vi "Main.vi"(11 "Module Admin":refnum<class "Delacor_lib_QMH_Cloneable Module Admin.lvclass">) -> ()   [LabVIEW 2026, in "Function Generator.lvlib"]
doc: "This template is based off of the Queued Message Handler design pattern and the Queued Message Handler project template that ships with LabVIEW.\n\nThe main difference is that the queue is private to this module and communication between modules is performed via Broadcast and Request events.\n\nRequest events are wrapped in public API methods and are handled in the Event Handling Loop (EHL) of this VI. Any module can register for Broadcast events sent by this module. The EHL generates messages based on user interface actions.\n\nThe Message Handling Loop (MHL) processes messages generated by the EHL, or by other messages. The messages are string values, so new messages can be added easily to the Message Cases case structure in the MHL. Each message cluster can also provide an optional value for Message Data, which is a variant that can be converted to whatever message-specific data is required.\n_____\nBased on DQMH Dev Tools: Project Template 7.1.2.1547."
uses:
  Function Generator.lvlib
  <vilib>/Delacor/Delacor QMH/Libraries/Cloneable Module Admin_class/Delacor_lib_QMH_Cloneable Module Admin.lvclass
  C:/Program Files/National Instruments/LabVIEW 2026/vi.lib/Delacor/Delacor QMH/Libraries/Module Admin_class/Delacor_lib_QMH_Module Admin.lvclass
  Module Data--cluster.ctl
  <vilib>/Delacor/Delacor QMH/Libraries/Cloneable Module Admin_class/Delacor_lib_QMH_Cloneable Module Admin.lvclass/Delacor_lib_QMH_Cloneable Module Admin.ctl
  Wake Up HL Argument--cluster.ctl
  <vilib>/Delacor/Delacor QMH/Libraries/Message Queue_class/Delacor_lib_QMH_Message Queue.lvclass/Delacor_lib_QMH_Message Queue.ctl
  Stop Argument--cluster.ctl
  <vilib>/Delacor/Delacor QMH/Libraries/Module Admin_class/Delacor_lib_QMH_Module Admin.lvclass/Delacor_lib_QMH_Module Admin.ctl
  Set Signal Type Argument--cluster.ctl
  Set Signal Parameters Argument--cluster.ctl
  Start Argument--cluster.ctl
  <vilib>/Utility/miscctls.llb/LVPointTypeDef.ctl
  <vilib>/Delacor/Delacor QMH/Libraries/Cloneable Module Admin_class/Delacor_lib_QMH_Get Module ID.vi
  <vilib>/Delacor/Delacor QMH/Libraries/Message Queue_class/Delacor_lib_QMH_Enqueue Message (Single).vi
  <vilib>/Delacor/Delacor QMH/Libraries/Module Admin_class/Delacor_lib_QMH_Get External Launch.vi
  <vilib>/Delacor/Delacor QMH/Libraries/Message Queue_class/Delacor_lib_QMH_Message Queue.lvclass
  <vilib>/measure/NI_MABase.lvlib
panel:
  out "error out":errorcluster
  out "Status":string
  in  "Simulate EHL Error":bool
  in  "Simulate MHL Error":bool
  # "Other processes communicate with this Module via its Public API (wrappers for its Request Events).\n\nThis Module communicates with other processes via its Broadcast Events.\nAny process that wants to receive these messages can register for this module's Broadcast events."
  # "This template is for the DQMH framework. See the block diagram for more information on how to use this template."
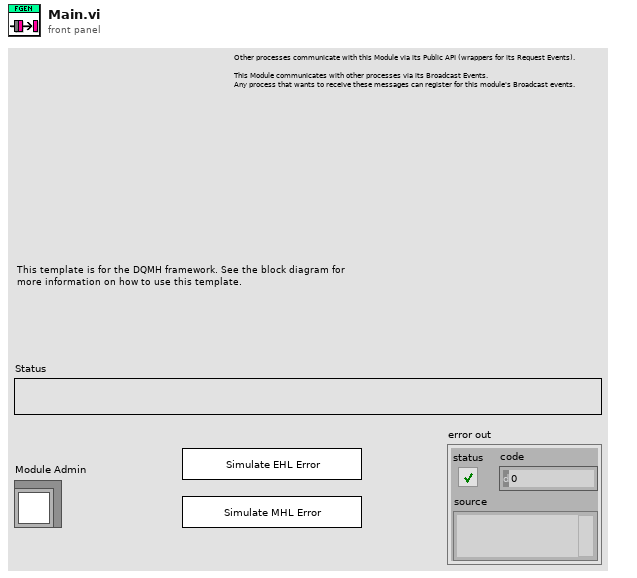
[diagram p1: front panel]
types:
  T1 = typedef "Function Generator.lvlib/Request Events--cluster.ctl" = cluster{"Stop Module":refnum<user-event>, "Show Panel":refnum<user-event>, "Hide Panel":refnum<user-event>, "Show Diagram":refnum<user-event>, "Get Module Execution Status":refnum<user-event>, "Set Signal Type":refnum<user-event>, "Set Signal Parameters":refnum<user-event>, "Start":refnum<user-event>, "Local Instance":T2, "Stop FGEN":refnum<user-event>}
  T2 = typedef "Function Generator.lvlib/Local Instance Request Events--cluster.ctl" = cluster{"Wake Up HL":refnum<user-event>}
  T3 = typedef "Function Generator.lvlib/Module Data--cluster.ctl" = cluster{"Status":string, "signal type":enum16{"Sine Wave", "Triangle Wave", "Square Wave", "Sawtooth Wave"}, "amplitude":dbl, "phase":dbl, "frequency":dbl, "offset 2":dbl}
  T4 = typedef "Function Generator.lvlib/Wake Up HL Argument--cluster.ctl" = cluster{"Module ID":i32, "Timeout":i32, "signal type":enum16{"Sine Wave", "Triangle Wave", "Square Wave", "Sawtooth Wave"}, "amplitude":dbl, "phase":dbl, "frequency":dbl, "offset 2":dbl}
  T5 = enum32{"invalid lock state", "Not Locked", "Locked (No Password)", "Password-protected"}
  T6 = typedef "Function Generator.lvlib/Stop Argument--cluster.ctl" = cluster{"Module ID":i32, "Origin":string, "Exit via Stop Module Req?":bool, "Wait for Module to stop?":bool}
  T7 = typedef "Function Generator.lvlib/Set Signal Type Argument--cluster.ctl" = cluster{"Module ID":i32, "signal type":enum16{"Sine Wave", "Triangle Wave", "Square Wave", "Sawtooth Wave"}}
  T8 = typedef "Function Generator.lvlib/Set Signal Parameters Argument--cluster.ctl" = cluster{"Module ID":i32, "amplitude":dbl, "phase":dbl, "frequency":dbl, "offset":dbl}
  T9 = typedef "Function Generator.lvlib/Start Argument--cluster.ctl" = cluster{"Module ID":i32, "Boolean":bool}
  T10 = typedef "LVPointTypeDef.ctl" = cluster{"Horizontal":i16, "Vertical":i16}
  T11 = enum32{"Invalid", "Standard", "Closed", "Hidden", "Minimized", "Maximized"}
  T12 = enum16{"Sine Wave", "Triangle Wave", "Square Wave", "Sawtooth Wave"}
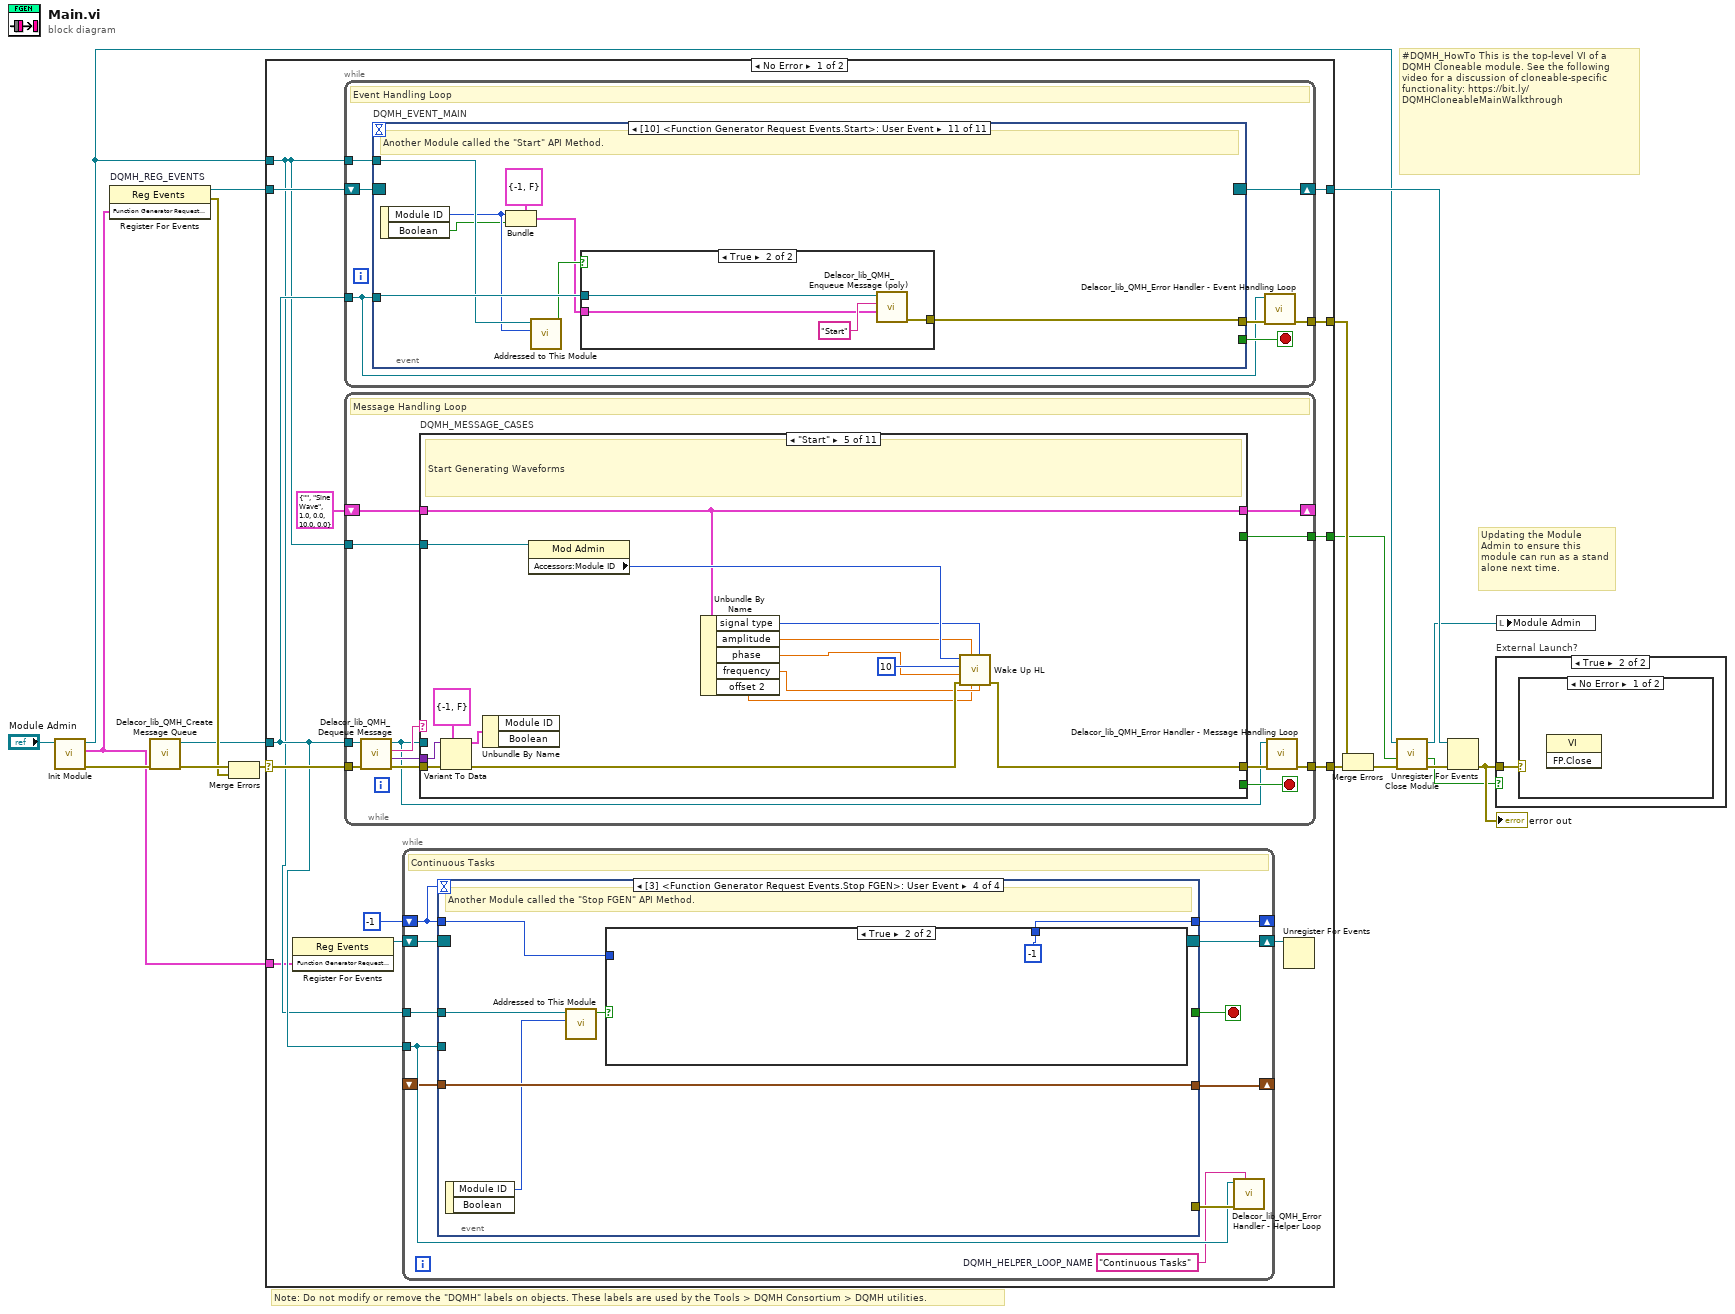
[diagram p0: block diagram]
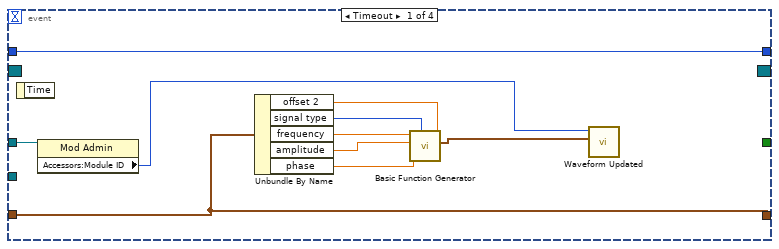
[diagram p2: hidden frame]
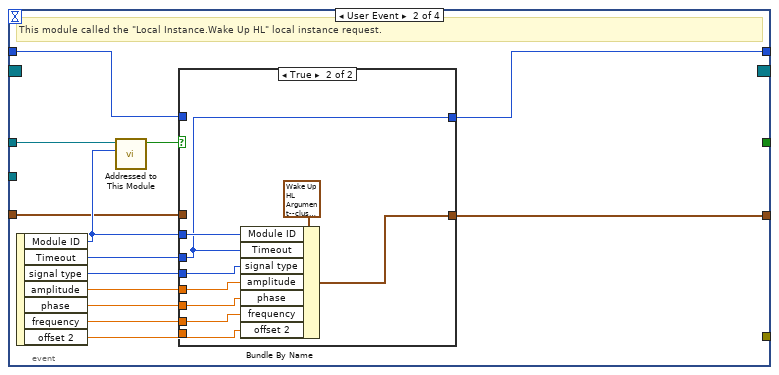
[diagram p3: hidden frame]
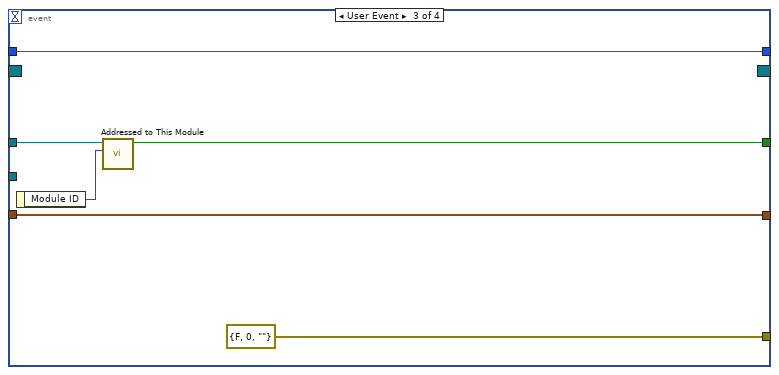
[diagram p5: hidden frame]
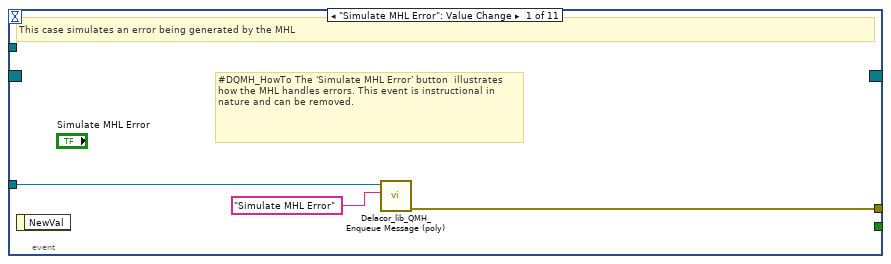
[diagram p7: hidden frame]
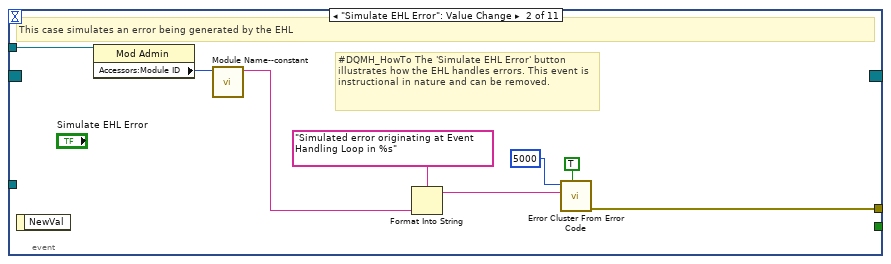
[diagram p8: hidden frame]
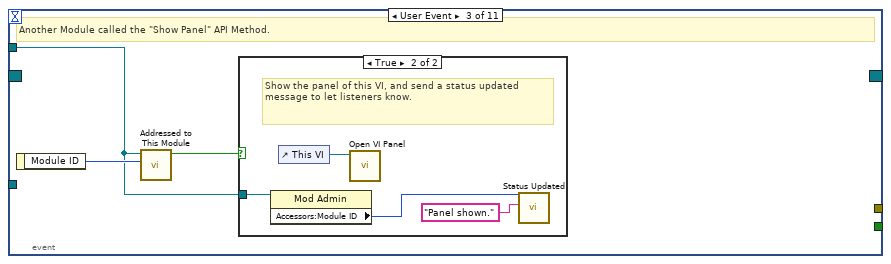
[diagram p9: hidden frame]
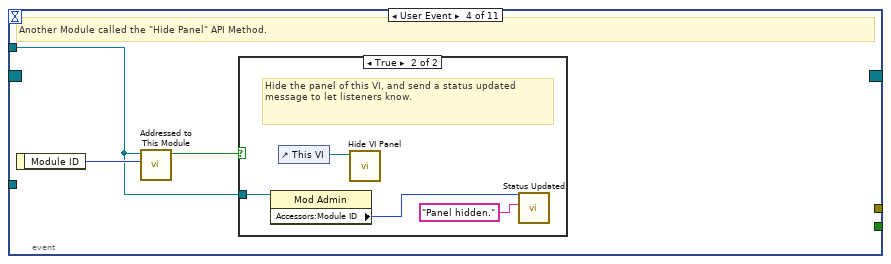
[diagram p11: hidden frame]
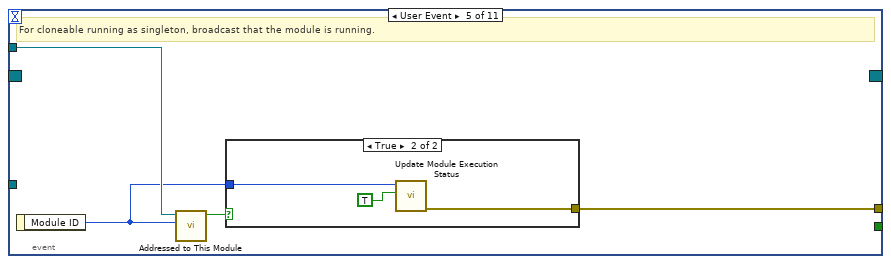
[diagram p13: hidden frame]
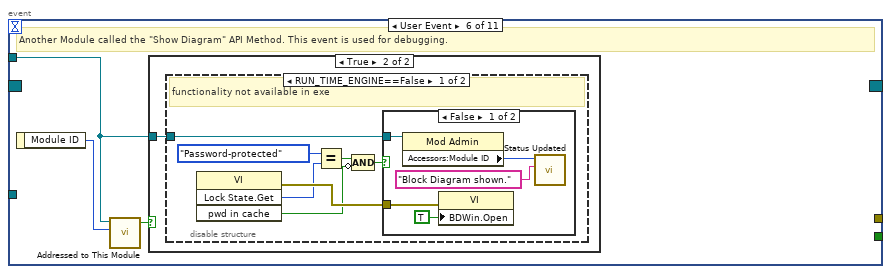
[diagram p15: hidden frame]
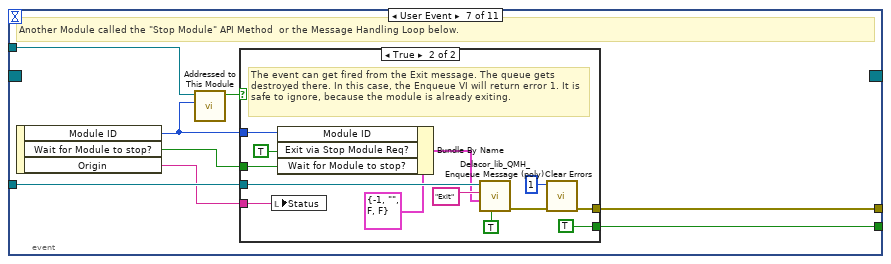
[diagram p19: hidden frame]
diagram:
  # "#DQMH_HowTo This is the top-level VI of a DQMH Cloneable module. See the following video for a discussion of cloneable-specific functionality: https://bit.ly/DQMHCloneableMainWalkthrough"
  # "Note: Do not modify or remove the \"DQMH\" labels on objects. These labels are used by the Tools > DQMH Consortium > DQMH utilities."
  # "Updating the Module Admin to ensure this module can run as a stand alone next time."
  n1 = call "Init Module.vi"("Cloneable Module Admin in"="Module Admin") -> ("error out"=w15:errorcluster, "Function Generator Request Events"=w1:T1, "Cloneable Module Admin out"=w5:refnum<class "Delacor_lib_QMH_Cloneable Module Admin.lvclass">)  [unwired: 8 in]
  n2 = register-events "DQMH_REG_EVENTS"(w1) -> (reference out=w8:refnum<event-registration>, error out=w10:errorcluster)  [unwired: 2 in]
  n3 = call <vilib>:"Delacor_lib_QMH_Create Message Queue.vi"("error in"=w15) -> ("error out"=w12:errorcluster, "Message Queue"=w7:refnum<class "Delacor_lib_QMH_Message Queue.lvclass">)  [unwired: 9 in]
  n4 = Merge Errors(w12, w10) -> (w11:errorcluster)
  n5 = case shown="No Error" w11 {
    selector: w11 -> [w29 w371]
    tunnel: [w31 w370] -> w16
    tunnel: [w28 w369] -> w9
    tunnel: w8 -> [w26 w369]
    tunnel: w7 -> [w25 w362]
    tunnel: [w30 _] -> w17
    tunnel: w5 -> [w24 w365]
    tunnel: [w23 _] -> w3
    tunnel: w1 -> [w22 _]
    frame No Error {
      n6 = register-events ("DQMH_HELPER_REGFOREVENTS")(w22) -> (reference out=w20:refnum<event-registration>)  [unwired: 2 in, 1 out]
      n7 = while {
        tunnel: w25 -> [w91]
        shift-right: [w94] -> w28
        shift-left: w26 -> [w95]
        tunnel: [w96] -> w30
        tunnel: w24 -> [w92]
        stop <- w93 stop-if-true
        # "Event Handling Loop"
        n8 = event "DQMH_EVENT_MAIN" shown="[10] <Function Generator Request Events.Start>: User Event" {
          selector: w95 -> [_ _ _ _ _ _ _ _ _ _ _]
          dyn-events: [_ _ _ _ _ _ _ _ _ _ _] -> w94
          timeout: _ -> [_ _ _ _ _ _ _ _ _ _ _]
          tunnel: [_ _ _ _ _ _ w149 _ _ _ _] -> w93
          tunnel: w91 -> [w99 _ _ _ _ _ w152 w169 w189 w204 w216]
          tunnel: [w100 w108 _ _ w126 _ w153 w172 w182 w194 w209] -> w97
          tunnel: w92 -> [_ w107 w109 w116 w124 w130 w151 w170 w187 w202 w214]
          event "Simulate MHL Error": Value Change {
            # "#DQMH_HowTo The 'Simulate MHL Error' button  illustrates how the MHL handles errors. This event is instructional in nature and can be removed."
            # "This case simulates an error being generated by the MHL"
            n9 = event-data() -> ()  [unwired: 1 in, 1 out]
            n10 = call-poly <vilib>:"Delacor_lib_QMH_Enqueue Message (poly).vi"("Message"="Simulate MHL Error", "Message Queue in"=w99) -> ("error out"=w100:errorcluster)  [unwired: 8 in, 1 out]
          }
          event "Simulate EHL Error": Value Change {
            # "#DQMH_HowTo The 'Simulate EHL Error' button  illustrates how the EHL handles errors. This event is instructional in nature and can be removed."
            # "This case simulates an error being generated by the EHL"
            n11 = event-data() -> ()  [unwired: 1 in, 1 out]
            n12 = property on="Property Node" class="Mod Admin"(reference=w107) -> ("Accessors:Module ID"=w106:i32)  [unwired: 1 in, 2 out]
            n13 = call "Module Name--constant.vi"("Module ID"=w106) -> ("Module Name"=w101:string)  [unwired: 10 in]
            n14 = Format Into String(format string="Simulated error originating at Event Handling Loop in %s", w101) -> (resulting string=w104:string)  [unwired: 2 in, 1 out]
            n15 = call <vilib>:"Error Cluster From Error Code.vi"("show call chain? (False)"=TRUE, "error message (\"\")"=w104, "error code (0)"=5000) -> ("error out"=w108:errorcluster)  [unwired: 6 in]
          }
          event User Event {
            # "Another Module called the \"Show Panel\" API Method."
            n16 = event-data() -> ("Module ID"=w110:i32)  [unwired: 1 in]
            n17 = call "Addressed to This Module.vi"("Module ID from Argument"=w110, "Module Admin"=w109) -> ("Addressed to this instance?"=w111:bool)  [unwired: 8 in, 1 out]
            n18 = case shown="True" w111 {
              tunnel: w109 -> [_ w113]
              frame False {
              }
              frame True {
                # "Show the panel of this VI, and send a status updated message to let listeners know."
                n19 = property on="Property Node" class="Mod Admin"(reference=w113) -> ("Accessors:Module ID"=w112:i32)  [unwired: 1 in, 2 out]
                n20 = control-ref of="This VI"() -> (w115:refnum<vi>)
                n21 = call "Open VI Panel.vi"("VI"=w115) -> ()  [unwired: 10 in, 1 out]
                n22 = call "Status Updated.vi"("Status"="Panel shown." ("format string"), "Module ID"=w112) -> ()  [unwired: 9 in, 1 out]
              }
            }
          }
          event User Event {
            # "Another Module called the \"Hide Panel\" API Method."
            n23 = event-data() -> ("Module ID"=w117:i32)  [unwired: 1 in]
            n24 = call "Addressed to This Module.vi"("Module ID from Argument"=w117, "Module Admin"=w116) -> ("Addressed to this instance?"=w118:bool)  [unwired: 8 in, 1 out]
            n25 = case shown="True" w118 {
              tunnel: w116 -> [_ w120]
              frame False {
              }
              frame True {
                # "Hide the panel of this VI, and send a status updated message to let listeners know."
                n26 = property on="Property Node" class="Mod Admin"(reference=w120) -> ("Accessors:Module ID"=w119:i32)  [unwired: 1 in, 2 out]
                n27 = control-ref of="This VI"() -> (w122:refnum<vi>)
                n28 = call "Hide VI Panel.vi"("VI"=w122) -> ()  [unwired: 10 in, 1 out]
                n29 = call "Status Updated.vi"("Status"="Panel hidden." ("format string"), "Module ID"=w119) -> ()  [unwired: 9 in, 1 out]
              }
            }
          }
          event User Event {
            # "For cloneable running as singleton, broadcast that the module is running."
            n30 = event-data() -> ("Module ID"=w123:i32)  [unwired: 1 in]
            n31 = call "Addressed to This Module.vi"("Module ID from Argument"=w123, "Module Admin"=w124) -> ("Addressed to this instance?"=w125:bool)  [unwired: 8 in, 1 out]
            n32 = case shown="True" w125 {
              tunnel: [_ w129] -> w126
              tunnel: w123 -> [_ w128]
              frame False {
              }
              frame True {
                n33 = call "Update Module Execution Status.vi"("Running?"=TRUE, "Module ID"=w128) -> ("error out"=w129:errorcluster)  [unwired: 9 in]
              }
            }
          }
          event User Event {
            # "Another Module called the \"Show Diagram\" API Method. This event is used for debugging."
            n34 = event-data() -> ("Module ID"=w131:i32)  [unwired: 1 in]
            n35 = call "Addressed to This Module.vi"("Module ID from Argument"=w131, "Module Admin"=w130) -> ("Addressed to this instance?"=w132:bool)  [unwired: 8 in, 1 out]
            n36 = case shown="True" w132 {
              tunnel: w130 -> [_ w133]
              frame False {
              }
              frame True {
                n37 = disable-structure shown="RUN_TIME_ENGINE==False" {
                  disable-tunnel: w133 -> [w134 _]
                  frame condition #0 (active) {
                    # "functionality not available in exe"
                    n38 = invoke on="Invoke Node" class="VI" method="Lock State.Get"() -> (error out=w140:errorcluster, "Get Lock State"=w139:T5, "pwd in cache"=w136:bool)  [unwired: 4 in, 1 out]
                    n39 = Equal?(x=T5."Password-protected", y=w139) -> (x = y?=w137:bool)
                    n40 = Compound Arithmetic op=AND(w137, invert w136) -> (w135:bool)
                    n41 = case shown="False" w135 {
                      tunnel: w140 -> [w145 _]
                      tunnel: w134 -> [w142 _]
                      frame False {
                        n42 = property on="Property Node" class="Mod Admin"(reference=w142) -> ("Accessors:Module ID"=w141:i32)  [unwired: 1 in, 2 out]
                        n43 = property on="Property Node" class="VI"(error in=w145, "BDWin.Open"=TRUE ("Block Diagram Window:Open")) -> ()  [unwired: 1 in, 2 out]
                        n44 = call "Status Updated.vi"("Status"="Block Diagram shown." ("format string"), "Module ID"=w141) -> ()  [unwired: 9 in, 1 out]
                      }
                      frame True {
                        # "Password-protected VI, and the password is not in the cache. Do not show the diagram."
                      }
                    }
                  }
                  frame condition #1 {
                  }
                }
              }
            }
          }
          event User Event {
            # "Another Module called the \"Stop Module\" API Method  or the Message Handling Loop below."
            n45 = event-data() -> ("Module ID"=w147:i32, "Wait for Module to stop?"=w148:bool, "Origin"=w146:string)  [unwired: 1 in]
            n46 = call "Addressed to This Module.vi"("Module ID from Argument"=w147, "Module Admin"=w151) -> ("Addressed to this instance?"=w150:bool)  [unwired: 8 in, 1 out]
            n47 = case shown="True" w150 {
              tunnel: [_ w165] -> w153
              tunnel: w152 -> [_ w161]
              tunnel: [_ TRUE] -> w149
              tunnel: w148 -> [_ w156]
              tunnel: w147 -> [_ w158]
              tunnel: w146 -> [_ w154]
              frame False {
              }
              frame True {
                # "The event can get fired from the Exit message. The queue gets destroyed there. In this case, the Enqueue VI will return error 1. It is safe to ignore, because the module is already exiting."
                n48 = local write "Status"(w154) -> ()
                n49 = Bundle By Name(cluster=T6 {"Module ID"=-1, "Origin"="", "Exit via Stop Module Req?"=FALSE, "Wait for Module to stop?"=FALSE} ("Stop Argument"), "Module ID"=w158, "Exit via Stop Module Req?"=TRUE, "Wait for Module to stop?"=w156) -> (w155:T6)
                n50 = call-poly <vilib>:"Delacor_lib_QMH_Enqueue Message (poly).vi"("Priority Message? (F)"=TRUE, "Message Data"=w155, "Message"="Exit", "Message Queue in"=w161) -> ("error out"=w166:errorcluster)  [unwired: 6 in, 1 out]
                n51 = call <vilib>:"Clear Errors.vi"("error in (no error)"=w166, "specific error code to clear (0: all)"=1) -> ("error out"=w165:errorcluster)  [unwired: 4 in, 1 out]
              }
            }
          }
          event Panel Close? {
            w171 = TRUE  # Discard the event, the MHL is responsible for closing and stopping this VI.
            # "Hide the panel or send the 'Exit' message if the user clicks the 'X' on the module main VI panel."
            n52 = event-data() -> ()  [unwired: 1 in, 1 out]
            n53 = property on="Property Node" class="Mod Admin"(reference=w170) -> (reference out=w167:refnum<class "Delacor_lib_QMH_Cloneable Module Admin.lvclass">, "Accessors:External Launch"=w168:bool)  [unwired: 1 in, 1 out]
            n54 = case shown="True" w168 {
              tunnel: w169 -> [_ w180]
              tunnel: [_ w181] -> w172
              tunnel: w167 -> [w175 _]
              frame True {
                # "If externally launched, clicking the 'X' hides the panel, but doesn't close it."
                n55 = property on="Property Node" class="Mod Admin"(reference=w175) -> ("Accessors:Module ID"=w174:i32)  [unwired: 1 in, 2 out]
                n56 = call "Status Updated.vi"("Status"="Panel hidden." ("format string"), "Module ID"=w174) -> ("error out"=w173:errorcluster)  [unwired: 9 in]
                n57 = control-ref of="This VI"() -> (w177:refnum<vi>)
                n58 = call "Hide VI Panel.vi"("error in"=w173, "VI"=w177) -> ()  [unwired: 9 in, 1 out]
              }
              frame False {
                # "If run as a stand-alone VI, clicking the panel 'X' stops the VI."
                n59 = call-poly <vilib>:"Delacor_lib_QMH_Enqueue Message (poly).vi"("Priority Message? (F)"=TRUE, "Message"="Exit", "Message Queue in"=w180) -> ("error out"=w181:errorcluster)  [unwired: 7 in, 1 out]
              }
            }
            n60 = event-data ("Event Filter Node")("Discard?"=w171) -> ()  [unwired: 1 in, 1 out]
          }
          event User Event {
            # "Another Module called the \"Set Signal Type\" API Method."
            n61 = event-data() -> ("Module ID"=w184:i32, "signal type"=w183:T12)  [unwired: 1 in]
            n62 = Bundle(cluster=T7 {"Module ID"=-1, "signal type"=enum."Sine Wave"} ("Set Signal Type Argument"), "Module ID"=w184, "signal type"=w183) -> (w185:T7)
            n63 = call "Addressed to This Module.vi"("Module ID from Argument"=w184, "Module Admin"=w187) -> ("Addressed to this instance?"=w188:bool)  [unwired: 8 in, 1 out]
            n64 = case shown="True" w188 {
              tunnel: w189 -> [_ w193]
              tunnel: w185 -> [_ w191]
              tunnel: [_ w190] -> w182
              frame False {
              }
              frame True {
                n65 = call-poly <vilib>:"Delacor_lib_QMH_Enqueue Message (poly).vi"("Message Data"=w191, "Message"="Set Signal Type", "Message Queue in"=w193) -> ("error out"=w190:errorcluster)  [unwired: 7 in, 1 out]
              }
            }
          }
          event User Event {
            # "Another Module called the \"Set Signal Parameters\" API Method."
            n66 = event-data() -> ("Module ID"=w199:i32, "amplitude"=w198:dbl, "phase"=w197:dbl, "frequency"=w196:dbl, "offset"=w195:dbl)  [unwired: 1 in]
            n67 = Bundle(cluster=T8 {"Module ID"=-1, "amplitude"=1.0, "phase"=0.0, "frequency"=10.0, "offset"=0.0} ("Set Signal Parameters Argument"), "Module ID"=w199, "amplitude"=w198, "phase"=w197, "frequency"=w196, "offset"=w195) -> (w200:T8)
            n68 = call "Addressed to This Module.vi"("Module ID from Argument"=w199, "Module Admin"=w202) -> ("Addressed to this instance?"=w203:bool)  [unwired: 8 in, 1 out]
            n69 = case shown="True" w203 {
              tunnel: w204 -> [_ w208]
              tunnel: w200 -> [_ w206]
              tunnel: [_ w205] -> w194
              frame False {
              }
              frame True {
                n70 = call-poly <vilib>:"Delacor_lib_QMH_Enqueue Message (poly).vi"("Message Data"=w206, "Message"="Set Signal Parameters", "Message Queue in"=w208) -> ("error out"=w205:errorcluster)  [unwired: 7 in, 1 out]
              }
            }
          }
          event User Event {
            # "Another Module called the \"Start\" API Method."
            n71 = event-data() -> ("Module ID"=w211:i32, "Boolean"=w210:bool)  [unwired: 1 in]
            n72 = Bundle(cluster=T9 {"Module ID"=-1, "Boolean"=FALSE} ("Start Argument"), "Module ID"=w211, "Boolean"=w210) -> (w212:T9)
            n73 = call "Addressed to This Module.vi"("Module ID from Argument"=w211, "Module Admin"=w214) -> ("Addressed to this instance?"=w215:bool)  [unwired: 8 in, 1 out]
            n74 = case shown="True" w215 {
              tunnel: w216 -> [_ w220]
              tunnel: w212 -> [_ w218]
              tunnel: [_ w217] -> w209
              frame False {
              }
              frame True {
                n75 = call-poly <vilib>:"Delacor_lib_QMH_Enqueue Message (poly).vi"("Message Data"=w218, "Message"="Start", "Message Queue in"=w220) -> ("error out"=w217:errorcluster)  [unwired: 7 in, 1 out]
              }
            }
          }
        }
        n76 = call-dynamic "Delacor_lib_QMH_Error Handler - Event Handling Loop.vi"("error in"=w97, "Message Queue in"=w91) -> ("dup error in"=w96:errorcluster)  [unwired: 8 in, 1 out]
      }
      n77 = while {
        tunnel: w25 -> [w221]
        shift-right: [w228] -> _
        shift-left: T3 {"Status"="", "signal type"=enum."Sine Wave", "amplitude"=1.0, "phase"=0.0, "frequency"=10.0, "offset 2"=0.0} ("Data Cluster") -> [w229]
        tunnel: w29 -> [w232]
        tunnel: [w230] -> w31
        tunnel: w24 -> [w223]
        tunnel: [w222] -> w23
        stop <- w227 stop-if-true
        # "Message Handling Loop"
        n78 = call-dynamic "Delacor_lib_QMH_Dequeue Message.vi"("error in"=w232, "Message Queue in"=w221) -> ("error out"=w231:errorcluster, "Message Data"=w225:variant, "Message"=w226:string, "Message Queue out"=w224:refnum<class "Delacor_lib_QMH_Message Queue.lvclass">)  [unwired: 6 in]
        n79 = case "DQMH_MESSAGE_CASES" shown="\"Start\"" w226 {
          selector: w226 -> [_ _ _ _ _ _ _ _ _ _ w351]
          tunnel: w224 -> [_ _ _ _ _ _ _ w306 _ w343 _]
          tunnel: w231 -> [w252 w256 w268 w283 w298 w301 w303 w315 w332 w349 w360]
          tunnel: [w250 w256 w266 w281 w292 w300 w303 w311 w331 w344 w361] -> w233
          tunnel: w229 -> [w243 w255 w267 w282 w289 w299 w302 w310 w329 w342 w358]
          tunnel: [w242 w255 w262 w277 w289 w299 w302 w310 w329 w342 w358] -> w228
          tunnel: [_ _ _ _ _ _ _ _ _ w341 _] -> w227
          tunnel: w225 -> [_ _ w265 w280 w297 _ _ w309 _ w339 _]
          tunnel: w223 -> [w238 _ w258 w274 w291 _ _ w308 w327 w334 w357]
          tunnel: [_ _ _ _ _ _ _ _ _ w337 _] -> w222
          frame "Initialize" {
            w235 = "Initial Message" ("Initial Message")
            # "#DQMH_CodeNeeded - Initialize the appearance of the front panel."
            # "#DQMH_CodeNeeded - Initialize your state data here."
            # "Initialize - Any operation that needs to be done before the module can receive messages. Synchronize Caller Events.vi will inform Start Module.vi that the module has launched and is ready to receive messages. Module Did Init.vi will broadcast that the module initialized."
            n80 = call "Synchronize Caller Events.vi"("error in"=w252, "Module Admin"=w238) -> ("error out"=w251:errorcluster, "Module Admin out"=w237:refnum<class "Delacor_lib_QMH_Cloneable Module Admin.lvclass">)  [unwired: 8 in]
            n81 = property on="Property Node" class="Mod Admin"(reference=w237) -> ("Accessors:Module ID"=w234:i32, "Accessors:External Launch"=w239:bool)  [unwired: 1 in, 2 out]
            n82 = call "Module Name--constant.vi"("Module ID"=w234) -> ("Module Name"=w247:string)  [unwired: 10 in]
            n83 = property on="Property Node" class="VI"("Front Panel.Title"=w247) -> (reference out=w249:refnum<vi>, error out=w254:errorcluster)  [unwired: 2 in]
            n84 = Select(t=T11."Hidden" ("State"), s=w239, f=T11."Standard" ("State")) -> (s? t:f=w244:T11)
            n85 = invoke on="Invoke Node" class="VI" method="FP.Open"(reference=w249, error in=w254, "State"=w244) -> (reference out=w248:refnum<vi>, error out=w253:errorcluster)  [unwired: 2 in, 3 out]
            n86 = Bundle By Name(cluster=w243, "Status"=w235) -> (w242:T3)
            n87 = invoke on="Invoke Node" class="VI" method="FP.Center"(reference=w248, error in=w253) -> ()  [unwired: 1 in, 3 out]
            n88 = property on="Pane" class="Pane"("Origin"=T10 {"Horizontal"=0, "Vertical"=0}) -> ()  [unwired: 2 in, 2 out]
            n89 = call "Module Name--constant.vi"("Module ID"=w234) -> ("Module Name"=w240:string)  [unwired: 10 in]
            n90 = call "Module Did Init.vi"("error in"=w251, "Initialized?"=TRUE, "Origin"=w240, "Module ID"=w234) -> ("error out"=w250:errorcluster)  [unwired: 7 in]
            "Status" <- w235
          }
          frame "---Module Specific---" {
            # "Separator -- The following cases handle messages specific to this Module."
          }
          frame "Set Signal Type" {
            # "Set Signal Type"
            n91 = Variant To Data(error in=w268, type=T7 {"Module ID"=-1, "signal type"=enum."Sine Wave"} ("Set Signal Type Argument"), Variant=w265) -> (data=w263:T7, error out=w266:errorcluster)
            n92 = property class="Mod Admin"(reference=w258) -> ("Accessors:Module ID"=w257:i32)  [unwired: 1 in, 2 out]
            n93 = Unbundle By Name(w263) -> ("signal type"=w261:T12)
            n94 = Bundle By Name(cluster=w267, "signal type"=w261) -> (w262:T3)
            n95 = Format Into String(format string="Signal type Selected: %s", w261) -> (resulting string=w260:string)  [unwired: 2 in, 1 out]
            n96 = call "Status Updated.vi"("Status"=w260, "Module ID"=w257) -> ()  [unwired: 9 in, 1 out]
          }
          frame "Set Signal Parameters" {
            n97 = Variant To Data(error in=w283, type=T8 {"Module ID"=-1, "amplitude"=1.0, "phase"=0.0, "frequency"=10.0, "offset"=0.0} ("Set Signal Parameters Argument"), Variant=w280) -> (data=w278:T8, error out=w281:errorcluster)
            n98 = Unbundle By Name(w278) -> ("amplitude"=w273:dbl, "phase"=w272:dbl, "frequency"=w271:dbl, "offset"=w270:dbl)
            n99 = property class="Mod Admin"(reference=w274) -> ("Accessors:Module ID"=w269:i32)  [unwired: 1 in, 2 out]
            n100 = Bundle By Name(cluster=w282, "amplitude"=w273, "phase"=w272, "frequency"=w271, "offset 2"=w270) -> (w277:T3)
            n101 = Format Into String(format string="Parameters Set: (Amplitude: %.2f, Phase: %.2f, Frecuency: %.2f, Offset: %.2f)", w273, w272, w271, w270) -> (resulting string=w276:string)  [unwired: 2 in, 1 out]
            n102 = call "Status Updated.vi"("Status"=w276, "Module ID"=w269) -> ()  [unwired: 9 in, 1 out]
          }
          frame "Start" {
            # "Start Generating Waveforms"
            n103 = Variant To Data(error in=w298, type=T9 {"Module ID"=-1, "Boolean"=FALSE} ("Start Argument"), Variant=w297) -> (data=w295:T9, error out=w293:errorcluster)
            n104 = Unbundle By Name(w295) -> ()  [unwired: 2 out]
            n105 = property class="Mod Admin"(reference=w291) -> ("Accessors:Module ID"=w294:i32)  [unwired: 1 in, 2 out]
            n106 = Unbundle By Name(w289) -> ("signal type"=w288:T12, "amplitude"=w287:dbl, "phase"=w286:dbl, "frequency"=w285:dbl, "offset 2"=w284:dbl)
            n107 = call "Wake Up HL.vi"("frequency"=w285, "signal type"=w288, "offset"=w284, "amplitude"=w287, "error in"=w293, "phase"=w286, "Timeout"=10, "Module ID"=w294) -> ("error out"=w292:errorcluster)  [unwired: 3 in]
          }
          frame "---Copy This Frame---" {
            # "Duplicate this frame when creating new messages.  Change this comment in the duplicated frame to describe this message."
            n108 = Merge Errors(w301) -> (w300:errorcluster)
          }
          frame "---Exit and Error Handling---" {
            # "Separator - the following cases handle errors and exit messages."
          }
          frame "Error" {
            # "#DQMH_CodeRecommended - If the module is running in standalone mode (External Launch = FALSE), this code will pop up an error dialog and call the 'Exit' message if an error occurs. Add more fine-grained error management here."
            # "Error - Check the error message data and respond accordingly. This message is sent by the \"Error Handler\" VIs at the end of each loop in this application."
            n109 = property on="Property Node" class="Mod Admin"(reference=w308) -> ("Accessors:External Launch"=w307:bool, "Accessors:Module ID"=w305:i32)  [unwired: 1 in, 2 out]
            n110 = Variant To Data(error in=w315, type=errorcluster {"status"=FALSE, "code"=0, "source"=""} ("error constant"), Variant=w309) -> (data=w304:errorcluster, error out=w313:errorcluster)
            n111 = local write "error out"(w304) -> ()
            n112 = call "Error Reported.vi"("Error"=w304, "Module ID"=w305) -> ()  [unwired: 9 in, 1 out]
            n113 = case shown="False" w307 {
              tunnel: [w320 _] -> w312
              tunnel: w306 -> [w318 _]
              tunnel: w304 -> [w319 _]
              frame False {
                n114 = disable-structure shown="Default" {
                  disable-tunnel: w319 -> [w321 _]
                  frame condition #0 (active) {
                    # "If the module is running standalone, then pop up an error dialog and call the \"Exit\" message."
                    n115 = call <vilib>:"Simple Error Handler.vi"("error in (no error)"=w321) -> ()  [unwired: 4 in, 5 out]
                  }
                  frame condition #1 {
                    # "To prevent the Simple Error Handler VI from being loaded (e.g. when deploying to a Real-Time target), add the Conditional Disable Symbol \"DQMH_Disable_SEH\" to your project and set it to TRUE."
                  }
                }
                n116 = call-poly <vilib>:"Delacor_lib_QMH_Enqueue Message (poly).vi"("Priority Message? (F)"=TRUE, "Message"="Exit", "Message Queue in"=w318) -> ("error out"=w320:errorcluster)  [unwired: 7 in, 1 out]
              }
              frame True {
                # "If the module was launched externally, calling the Error Reported broadcast VI is the only action performed by the \"Error\" message. The module's caller can then process the error appropriately."
              }
            }
            n117 = Merge Errors(w313, w312) -> (w311:errorcluster)
          }
          frame "Simulate MHL Error" {
            # "#DQMH_HowTo The 'Simulate MHL Error' button  illustrates how the MHL handles errors. This event is instructional in nature and can be removed."
            # "Simulate an error occurring at the MHL"
            n118 = property on="Property Node" class="Mod Admin"(reference=w327) -> ("Accessors:Module ID"=w328:i32)  [unwired: 1 in, 2 out]
            n119 = call "Module Name--constant.vi"("Module ID"=w328) -> ("Module Name"=w323:string)  [unwired: 10 in]
            n120 = Format Into String(format string="Simulated error originating at Message Handling Loop in %s", w323) -> (resulting string=w324:string)  [unwired: 2 in, 1 out]
            n121 = call <vilib>:"Error Cluster From Error Code.vi"("show call chain? (False)"=TRUE, "error message (\"\")"=w324, "error code (0)"=5001) -> ("error out"=w330:errorcluster)  [unwired: 6 in]
            n122 = Merge Errors(w332, w330) -> (w331:errorcluster)
          }
          frame "Exit" {
            w340 = 91  # 91: not all Exit messages will have an argument
            w341 = TRUE  # Stop the VI
            # "Release the message queue reference"
            # "#DQMH_CodeNeeded - Add any required cleanup code here."
            # "Exit - Exit the application."
            n123 = Variant To Data(error in=w349, type=T6 {"Module ID"=-1, "Origin"="", "Exit via Stop Module Req?"=FALSE, "Wait for Module to stop?"=FALSE} ("Stop Argument"), Variant=w339) -> (data=w336:T6, error out=w345:errorcluster)
            n124 = call <vilib>:"Clear Errors.vi"("error in (no error)"=w345, "specific error code to clear (0: all)"=w340) -> ("error out"=w348:errorcluster)  [unwired: 4 in, 1 out]
            n125 = property on="Property Node" class="Mod Admin"(reference=w334) -> ("Accessors:Module ID"=w333:i32)  [unwired: 1 in, 2 out]
            n126 = control-ref of="This VI"() -> (w335:refnum<vi>)
            n127 = call-dynamic "Delacor_lib_QMH_Release Message Queue.vi"("error in"=w348, "Message Queue"=w343) -> ("error out"=w347:errorcluster)  [unwired: 9 in]
            n128 = call "Handle Exit.vi"("Stop Argument"=w336, "Module Admin in"=w334, "VI reference"=w335) -> ("error out"=w346:errorcluster, "Wait for Stop?"=w337:bool)  [unwired: 7 in]
            n129 = Merge Errors(w347, w346) -> (w344:errorcluster)
            n130 = call "Error Reported.vi"("Error"=w344, "Module ID"=w333) -> ()  [unwired: 9 in, 1 out]
          }
          frame Default {
            # "'Default' case only runs if there is a message that isn't defined in any of the other cases.  Output a programming error."
            n131 = property on="Property Node" class="Mod Admin"(reference=w357) -> ("Accessors:Module ID"=w356:i32)  [unwired: 1 in, 2 out]
            n132 = call "Module Name--constant.vi"("Module ID"=w356) -> ("Module Name"=w350:string)  [unwired: 10 in]
            n133 = Format Into String(format string="The invalid message string \"%s\" was received in the Message Handling Loop for module \"%s\".", w351, w350) -> (resulting string=w353:string)  [unwired: 2 in, 1 out]
            n134 = call <vilib>:"Error Cluster From Error Code.vi"("show call chain? (False)"=TRUE, "error message (\"\")"=w353, "error code (0)"=1) -> ("error out"=w359:errorcluster)  [unwired: 6 in]
            n135 = Merge Errors(w360, w359) -> (w361:errorcluster)
          }
        }
        n136 = call-dynamic "Delacor_lib_QMH_Error Handler - Message Handling Loop.vi"("error in"=w233, "Message Queue in"=w224) -> ("dup error in"=w230:errorcluster)  [unwired: 8 in, 1 out]
      }
      n137 = while "DQMH_HELPER_LOOP" {
        shift-right: [w42] -> _
        shift-left: -1 -> [w41]
        shift-right: [w39] -> w21
        shift-left: w20 -> [w40]
        tunnel: w25 -> [w36]
        tunnel: w24 -> [w34]
        shift-right: [w33] -> _
        shift-left: _ -> [w32]
        stop <- w38 stop-if-true
        w35 = "Continuous Tasks"  # DQMH_HELPER_LOOP_NAME
        # "Continuous Tasks"
        n138 = event "DQMH_HELPER_EVENT_STRUCTURE" shown="[3] <Function Generator Request Events.Stop FGEN>: User Event" {
          selector: w40 -> [_ _ _ _]
          dyn-events: [_ _ _ _] -> w39
          timeout: w41 -> [_ _ _ _]
          tunnel: w41 -> [w52 w55 w82 w84]
          tunnel: [w52 w56 w82 w83] -> w42
          tunnel: [_ _ w79 _] -> w38
          tunnel: [_ _ errorcluster {"status"=FALSE, "code"=0, "source"=""} ("error constant") _] -> w37
          tunnel: w36 -> [_ _ _ _]
          tunnel: w34 -> [w44 w65 w80 w87]
          tunnel: [w51 w54 w77 w88] -> w33
          tunnel: w32 -> [w51 w53 w77 w88]
          event Timeout {
            n139 = event-data() -> ()  [unwired: 1 in, 1 out]
            n140 = property class="Mod Admin"(reference=w44) -> ("Accessors:Module ID"=w43:i32)  [unwired: 1 in, 2 out]
            n141 = Unbundle By Name(w51) -> ("offset 2"=w49:dbl, "signal type"=w50:T12, "frequency"=w48:dbl, "amplitude"=w47:dbl, "phase"=w46:dbl)
            n142 = call <vilib>:"Basic Function Generator.vi"("offset"=w49, "signal type"=w50, "phase"=w46, "amplitude"=w47, "frequency"=w48) -> ("signal out"=w45:waveform(dbl))  [unwired: 4 in, 2 out]
            n143 = call "Waveform Updated.vi"("signal out"=w45, "Module ID"=w43) -> ()  [unwired: 9 in, 1 out]
          }
          event User Event {
            # "This module called the \"Local Instance.Wake Up HL\" local instance request."
            n144 = event-data() -> ("Module ID"=w64:i32, "Timeout"=w63:i32, "signal type"=w62:T12, "amplitude"=w61:dbl, "phase"=w60:dbl, "frequency"=w59:dbl, "offset 2"=w58:dbl)  [unwired: 1 in]
            n145 = call "Addressed to This Module.vi"("Module ID from Argument"=w64, "Module Admin"=w65) -> ("Addressed to this instance?"=w57:bool)  [unwired: 8 in, 1 out]
            n146 = case shown="True" w57 {
              tunnel: w64 -> [_ w75]
              tunnel: w63 -> [_ w69]
              tunnel: w62 -> [_ w74]
              tunnel: w61 -> [_ w73]
              tunnel: w60 -> [_ w72]
              tunnel: w59 -> [_ w71]
              tunnel: w58 -> [_ w70]
              tunnel: [w67 w69] -> w56
              tunnel: w55 -> [w67 _]
              tunnel: [w66 w68] -> w54
              tunnel: w53 -> [w66 _]
              frame False {
              }
              frame True {
                n147 = Bundle By Name(cluster=T4 {"Module ID"=-1, "Timeout"=0, "signal type"=enum."Sine Wave", "amplitude"=1.0, "phase"=0.0, "frequency"=10.0, "offset 2"=0.0}, "Module ID"=w75, "Timeout"=w69, "signal type"=w74, "amplitude"=w73, "phase"=w72, "frequency"=w71, "offset 2"=w70) -> (w68:T4)
              }
            }
          }
          event User Event {
            n148 = event-data() -> ("Module ID"=w78:i32)  [unwired: 1 in]
            n149 = call "Addressed to This Module.vi"("Module ID from Argument"=w78, "Module Admin"=w80) -> ("Addressed to this instance?"=w79:bool)  [unwired: 8 in, 1 out]
          }
          event User Event {
            # "Another Module called the \"Stop FGEN\" API Method."
            n150 = event-data() -> ("Module ID"=w86:i32)  [unwired: 1 in, 1 out]
            n151 = call "Addressed to This Module.vi"("Module ID from Argument"=w86, "Module Admin"=w87) -> ("Addressed to this instance?"=w85:bool)  [unwired: 8 in, 1 out]
            n152 = case shown="True" w85 {
              tunnel: w84 -> [w89 _]
              tunnel: [w89 -1 ("Timeout")] -> w83
              frame False {
              }
              frame True {
              }
            }
          }
        }
        n153 = call-dynamic "Delacor_lib_QMH_Error Handler - Helper Loop.vi"("Error Debug"=w35, "error in"=w37, "Message Queue in"=w36) -> ()  [unwired: 7 in, 2 out]
      }
      n154 = Unregister For Events(event registration refnum=w21) -> ()  [unwired: 1 in, 1 out]
    }
    frame Error {
      n155 = call "Synchronize Caller Events.vi"("Module Admin"=w365) -> ("Module Admin out"=w364:refnum<class "Delacor_lib_QMH_Cloneable Module Admin.lvclass">)  [unwired: 9 in, 1 out]
      n156 = property on="Property Node" class="Mod Admin"(reference=w364) -> ("Accessors:Module ID"=w363:i32)  [unwired: 1 in, 2 out]
      n157 = call-dynamic "Delacor_lib_QMH_Release Message Queue.vi"("error in"=w371, "Message Queue"=w362) -> ("error out"=w370:errorcluster)  [unwired: 9 in]
      n158 = call "Module Name--constant.vi"("Module ID"=w363) -> ("Module Name"=w368:string)  [unwired: 10 in]
      n159 = Format Into String(format string="An error occurred during initialization. %s is no longer running.", w368) -> (resulting string=w366:string)  [unwired: 2 in, 1 out]
      n160 = call "Error Reported.vi"("Additional Information"=w366, "Error"=w370, "Module ID"=w363) -> ()  [unwired: 8 in, 1 out]
    }
  }
  n161 = Merge Errors(w17, w16) -> (w18:errorcluster)
  n162 = call "Close Module.vi"("error in"=w18, "Wait for stop?"=w3, "Module Admin in"=w5) -> ("error out"=w14:errorcluster, "External Launch"=w2:bool, "Module Admin out"=w4:refnum<class "Delacor_lib_QMH_Cloneable Module Admin.lvclass">)  [unwired: 6 in]
  n163 = Unregister For Events(event registration refnum=w9, error in=w14) -> (error out=w13:errorcluster)
  "error out" <- w13
  n164 = case "External Launch?" shown="True" w2 {
    tunnel: w13 -> [_ w372]
    frame False {
    }
    frame True {
      n165 = case shown="No Error" w372 {
        frame No Error {
          n166 = invoke class="VI" method="FP.Close"() -> ()  [unwired: 3 in, 3 out]
        }
        frame Error {
          n167 = disable-structure shown="Default" {
            frame condition #0 (active) {
              n168 = invoke class="VI" method="FP.Open"("Activate"=TRUE ("Activate?")) -> ()  [unwired: 4 in, 5 out]
            }
            frame condition #1 {
              # "Don't show panel on error if running inside a built EXE."
            }
          }
        }
      }
    }
  }
  n169 = local write "Module Admin"(w4) -> ()
